vi "[ex ce] 3 Passing parameters via variables.vi"() -> ()   [LabVIEW 2021]
doc: "<B>Passing parameters via variables</B> (CE Client Example)\n\nThis simple example shows how you can pass parameters to CE Server via variables. Similar to this example, you can pass parameters of any type supported by CalcExpress.\n\nTo execute this example, you need run <B>[ex ce] CE Server Example.vi</B> on either local or remote computer. Also, you need <B>LabVIEW Advanced Analysis VIs</B> on server side.\n\n::: CalcExpress Toolkit :::\nCopyright (c) 2000-2026 Konstantin Shifershteyn. All rights reserved."
panel:
  in  "Periods":cluster{"name":string, "value":dbl}={"name"="Cycles", "value"=3.0} caption="Cycles" {"value" min=1.0 max=8.0 scale=0.0..8.0}
  in  "Amp":cluster{"name":string, "value":dbl}={"name"="Amp", "value"=7.5} caption="Amplitude" {"value" min=0.0 max=10.0 scale=0.0..10.0 scale format="%.1f"}
  in  "Ns":cluster{"name":string, "value":u32}={"name"="Ns", "value"=1000} caption="Number of samples"
  in  "stop":bool
  in  "To execute this example, you need run \"[ex ce] CE Server Example.vi\" on either local or remote computer. Also, you need the Advanced Analysis Libraries on server side.\n-------------------------------------------\nThis simple example demonstrates how you can pass parameters to CE Server via variables. Similar to this example, you can pass parameters of any data type supported by CalcExpress.":string="To execute this example, you need run \"[ex ce] CE Server Example.vi\" on either local or remote computer. Also, you need the Advanced Analysis Libraries on server side.\n-------------------------------------------\nThis simple example demonstrates how you can pass parameters to CE Server via variables. Similar to this example, you can pass parameters of any data type supported by CalcExpress."
  in  "use TCP for local":bool
  in  "expression":string="base = pSine(Ns, 1, 0, 100);\npSine(Ns, Amp, 0, Cycles/2) * base\n"
  out "graph":dbl[](graph)
  in  "port":u32=3363
  in  "machine name (empty - local)":string
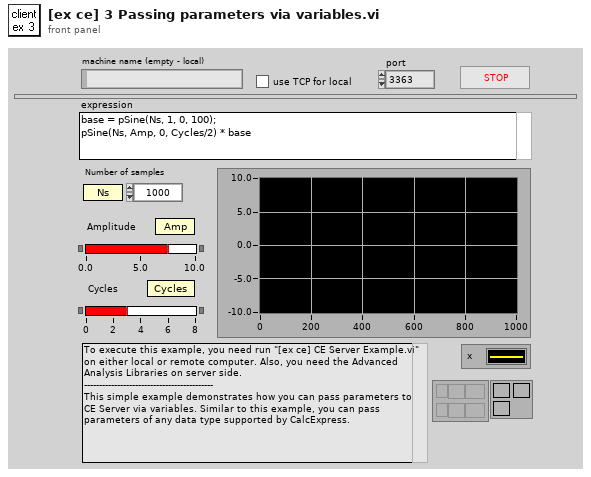
[diagram p1: front panel]
types:
  T1 = typedef "CE Session.ctl" = cluster{"VI refnum":refnum<vi>, "VC Handle":T2}
  T2 = typedef "VarMan Variable Context Handle.ctl" = i32
  T3 = cluster{"type":enum32{"String", "DBL Number", "identifier", "1D Array of DBL", "2D Array of DBL", "CDB Number", "1D Array of CDB", "2D Array of CDB", "1D Array of String", "2D Array of String", "Unknown data type"}, "dbl":dbl, "cdb":cdb, "str":string, "1d dbl":dbl[], "1d cdb":cdb[], "1d str":string[], "2d dbl":dbl[][], "2d cdb":cdb[][], "2d str":string[][]}
  T4 = enum16{"create", "destroy", "set value", "get value"}
  T5 = enum32{"String", "DBL Number", "identifier", "1D Array of DBL", "2D Array of DBL", "CDB Number", "1D Array of CDB", "2D Array of CDB", "1D Array of String", "2D Array of String", "Unknown data type"}
  T6 = typedef "CalcExpress Data Type.ctl" = enum32{"String", "DBL Number", "identifier", "1D Array of DBL", "2D Array of DBL", "CDB Number", "1D Array of CDB", "2D Array of CDB", "1D Array of String", "2D Array of String", "Unknown data type"}
  T7 = cluster{"type":T6, "dbl":dbl, "cdb":cdb, "str":string, "1d dbl":dbl[], "1d cdb":cdb[], "1d str":string[], "2d dbl":dbl[][], "2d cdb":cdb[][], "2d str":string[][]}
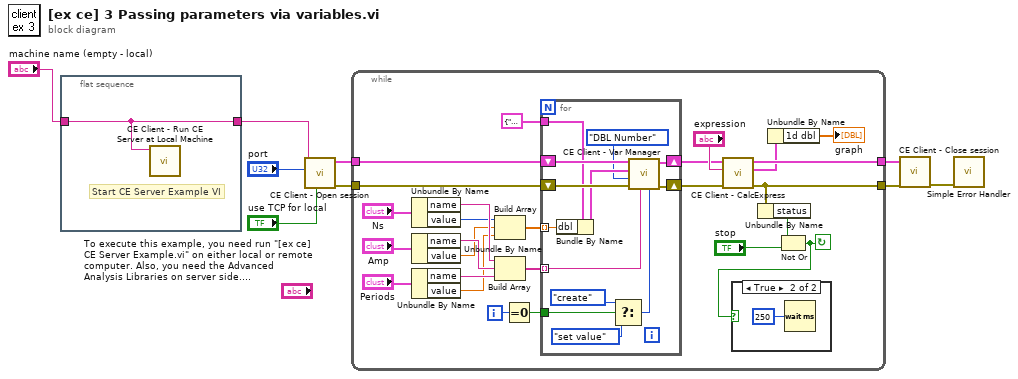
[diagram p0: block diagram]
diagram:
  n1 = flat-sequence {
    tunnel: [w10] -> w1
    tunnel: "machine name (empty - local)" -> [w10]
    frame #0 {
      # "Start CE Server Example VI"
      n2 = call "CE Client - Run CE Server at Local Machine.vi"("machine name"=w10) -> ()  [unwired: 9 in, 2 out]
    }
  }
  n3 = call "CE Client - Open session.vi"("use TCP for local (F)"="use TCP for local", "port number (3363)"="port", "machine name (empty - local)"=w1) -> ("error out"=w5:errorcluster, "CE session out"=w6:T1)  [unwired: 5 in]
  n4 = while {
    tunnel: [w29] -> w3
    tunnel: [w30] -> w4
    tunnel: w5 -> [w31]
    tunnel: w6 -> [w32]
    i -> [w17]
    stop <- w13 continue-if-true
    n5 = Unbundle By Name("Ns") -> ("name"=w23:string, "value"=w18:u32)
    n6 = Unbundle By Name("Amp") -> ("name"=w22:string, "value"=w19:dbl)
    n7 = Unbundle By Name("Periods") -> ("name"=w21:string, "value"=w20:dbl)
    n8 = Build Array(w18, w19, w20) -> (w14:dbl[])
    n9 = Build Array(w23, w22, w21) -> (w15:string[])
    n10 = Equal To 0?(x=w17) -> (x = 0?=w16:bool)
    n11 = for {
      shift-right: [w47] -> w33
      shift-left: w31 -> [w50]
      shift-right: [w48] -> w34
      shift-left: w32 -> [w49]
      tunnel: w16 -> [w43]
      tunnel: w15 -> [w42] mode=indexing
      tunnel: w14 -> [w41] mode=indexing
      tunnel: T3 {"type"=enum."DBL Number", "dbl"=0.0, "cdb"=0.0+0.0i, "str"="", "1d dbl"=[], "1d cdb"=[], "1d str"=[], "2d dbl"=[], "2d cdb"=[], "2d str"=[]} ("values in") -> [w40]
      n12 = Bundle By Name(cluster=w40, "dbl"=w41) -> (w39:T3)
      n13 = Select(t=T4."create" ("var cmd"), s=w43, f=T4."set value" ("var cmd")) -> (s? t:f=w46:T4)
      n14 = call "CE Client - Var Manager.vi"("var cmd"=w46, "var name"=w42, "error in"=w50, "var type"=T5."DBL Number" ("data type"), "values in"=w39, "CE session"=w49) -> ("error out"=w47:errorcluster, "dup CE session"=w48:T1)  [unwired: 1 in, 1 out]
    }
    n15 = call "CE Client - CalcExpress.vi"("error in"=w33, "expression"="expression", "CE session"=w34) -> ("error out"=w29:errorcluster, "values out"=w12:T7, "dup CE session"=w30:T1)  [unwired: 4 in]
    n16 = Unbundle By Name(w29) -> ("status"=w28:bool)
    n17 = Unbundle By Name(w12) -> ("1d dbl"=→"graph":dbl[])
    n18 = Not Or(1:"stop", 2:w28) -> (0:w13:bool)
    n19 = case shown="True" w13 {
      frame False {
      }
      frame True {
        n20 = Wait (ms)(milliseconds to wait=u32 250) -> ()  [unwired: 1 out]
      }
    }
  }
  n21 = call "CE Client - Close session.vi"("error in"=w3, "CE session"=w4) -> ("error out"=w8:errorcluster)  [unwired: 6 in, 1 out]
  n22 = call <vilib>:"Simple Error Handler.vi"("error in (no error)"=w8) -> ()  [unwired: 4 in, 5 out]
